vi "VIH Dialog - Search Files in Folder.vi"(8 "error in":errorcluster, 9 "File Paths":path[](array[path]), 10 "Tree Item Tags":string[](array[string]), 11 "Project Tree":T1) -> (0 "error out":errorcluster, 1 "File Paths out":path[](array[path]), 2 "Tree Item Tags out":string[](array[string]), 3 "dup Project Tree":T1)   [LabVIEW 2014]
doc: "::: VI Helpeks :::\nCopyright (c) 2000-2026 Konstantin Shifershteyn. All rights reserved."
uses:
  VIH Project Tree Typedef - Tree Refnum.ctl
panel:
  # "VI Helpeks\nCopyright (c) 2012-2026 Konstantin Shifershteyn"
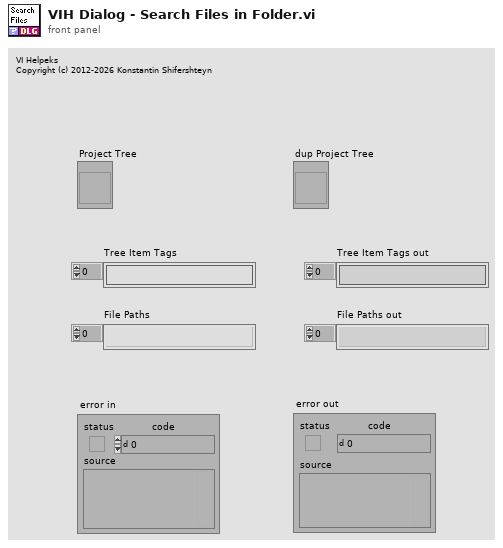
[diagram p1: front panel]
types:
  T1 = typedef "VIH Project Tree Typedef - Tree Refnum.ctl" = refnum<vi>
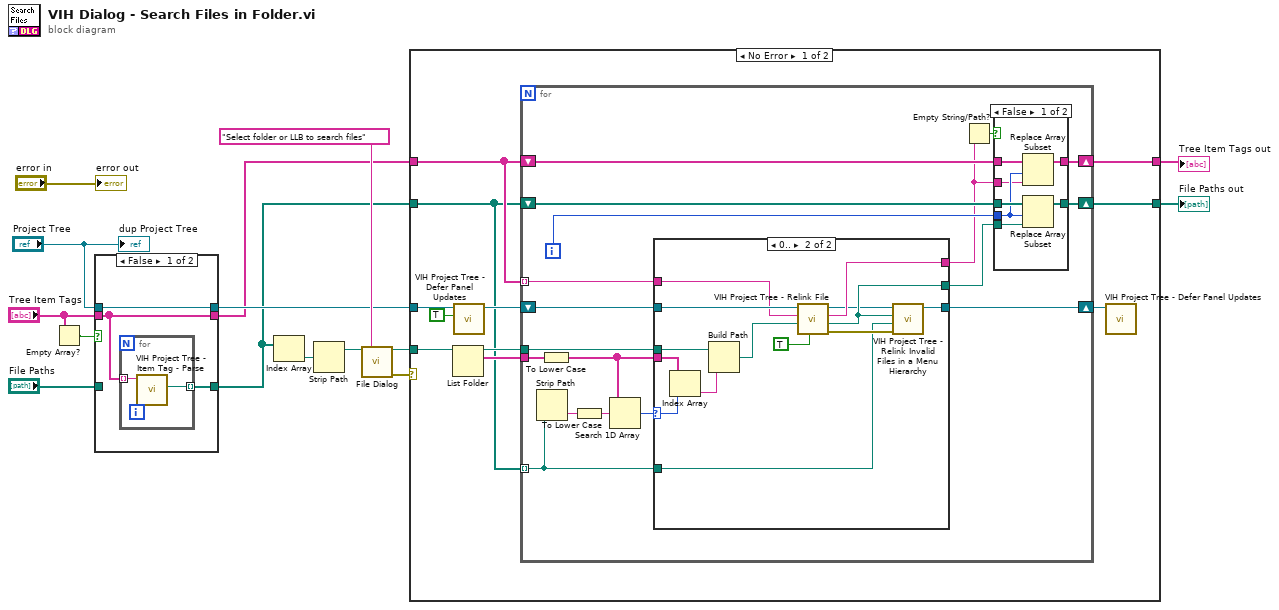
[diagram p0: block diagram]
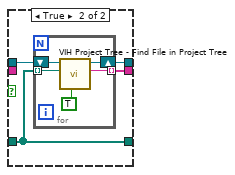
[diagram p2: hidden frame]
diagram:
  n1 = Empty Array?(array="Tree Item Tags") -> (empty?=w10:bool)
  n2 = case shown="False" w10 {
    tunnel: [w18 w24] -> w4
    tunnel: "Tree Item Tags" -> [w18 _]
    tunnel: [w17 w23] -> w3
    tunnel: "File Paths" -> [_ w23]
    tunnel: "Project Tree" -> [w16 w22]
    tunnel: [w16 w21] -> w6
    frame False {
      n3 = for {
        tunnel: w18 -> [w20] mode=indexing
        tunnel: [w19] -> w17 mode=indexing
        n4 = call "VIH Project Tree - Item Tag - Parse.vi"("Tree Item Tag"=w20) -> ("Item File Path"=w19:path)  [unwired: 8 in, 2 out]
      }
    }
    frame True {
      n5 = for {
        tunnel: [w28] -> w24 mode=indexing
        tunnel: w23 -> [w27] mode=indexing
        shift-right: [w25] -> w21
        shift-left: w22 -> [w26]
        n6 = call "VIH Project Tree - Find File in Project Tree.vi"("Ena <Invalid> (F)"=TRUE, "File Path"=w27, "Project Tree"=w26) -> ("Tree Item Tag (Static)"=w28:string, "dup Project Tree"=w25:T1)  [unwired: 5 in, 2 out]
      }
    }
  }
  n7 = Index Array(array=w3) -> (element=w5:path)  [unwired: 1 in]
  n8 = Strip Path(path=w5) -> (stripped path=w14:path)  [unwired: 1 out]
  n9 = call "File Dialog"("start path"=w14, "prompt"="Select folder or LLB to search files") -> ("selected path"=w13:path, "error out"=w12:errorcluster)  [unwired: 10 in, 2 out]
  n10 = case shown="No Error" w12 {
    tunnel: w6 -> [w40 _]
    tunnel: w13 -> [w36 _]
    tunnel: w4 -> [w33 _]
    tunnel: w3 -> [w32 _]
    tunnel: [w31 _] -> w2
    tunnel: [w30 _] -> w1
    frame No Error {
      n11 = List Folder(path=w36) -> (path out=w34:path, filenames=w35:string[])  [unwired: 3 in, 2 out]
      n12 = call "VIH Project Tree - Defer Panel Updates.vi"("Defer Panel Updates (F)"=TRUE, "Project Tree"=w40) -> ("dup Project Tree"=w39:T1)  [unwired: 7 in, 2 out]
      n13 = for {
        tunnel: w32 -> [w56] mode=indexing
        shift-right: [w57] -> w38
        shift-left: w39 -> [w58]
        tunnel: w35 -> [w54]
        tunnel: w33 -> [w52] mode=indexing
        tunnel: w34 -> [w50]
        shift-right: [w46] -> w31
        shift-left: w33 -> [w48]
        shift-right: [w45] -> w30
        shift-left: w32 -> [w47]
        i -> [w44]
        n14 = Strip Path(path=w56) -> (name=w55:string)  [unwired: 1 out]
        n15 = To Lower Case(string=w54) -> (all lower case string=w49:string[])
        n16 = To Lower Case(string=w55) -> (all lower case string=w53:string)
        n17 = Search 1D Array(1D array=w49, element=w53) -> (index of element=w51:i32)  [unwired: 1 in]
        n18 = case shown="0.." w51 {
          selector: w51 -> [_ w71]
          tunnel: [_ w82] -> w43
          tunnel: [_ w81] -> w42
          tunnel: w58 -> [w68 w77]
          tunnel: [w68 w76] -> w57
          tunnel: w56 -> [_ w75]
          tunnel: w52 -> [_ w74]
          tunnel: w50 -> [_ w73]
          tunnel: w49 -> [_ w72]
          frame ..-1 {
          }
          frame 0.. {
            n19 = Index Array(array=w72, index=w71) -> (element=w70:string)
            n20 = Build Path(base path=w73, name or relative path=w70) -> (appended path=w69:path)
            n21 = call "VIH Project Tree - Relink File.vi"("Ena Dialog Message (T)"=TRUE, "New File Path"=w69, "Tree Item Tag"=w74, "Project Tree"=w77) -> ("error out"=w78:errorcluster, "New File Path out"=w81:path, "New Tree Item Tag"=w82:string, "dup Project Tree"=w80:T1)  [unwired: 4 in]
            n22 = call "VIH Project Tree - Relink Invalid Files in a Menu Hierarchy.vi"("error in"=w78, "old Item Path"=w75, "new Item Path"=w81, "Project Tree"=w80) -> ("dup Project Tree"=w76:T1)  [unwired: 6 in, 1 out]
          }
        }
        n23 = Empty String/Path?(string/path=w43) -> (empty?=w41:bool)
        n24 = case shown="False" w41 {
          tunnel: w48 -> [w65 w67]
          tunnel: w47 -> [w64 w66]
          tunnel: [w63 w67] -> w46
          tunnel: [w62 w66] -> w45
          tunnel: w44 -> [w61 _]
          tunnel: w43 -> [w60 _]
          tunnel: w42 -> [w59 _]
          frame False {
            n25 = Replace Array Subset(array=w65, new element=w60, index=w61) -> (w63:string[])
            n26 = Replace Array Subset(array=w64, new element=w59, index=w61) -> (w62:path[])
          }
          frame True {
          }
        }
      }
      n27 = call "VIH Project Tree - Defer Panel Updates.vi"("Project Tree"=w38) -> ()  [unwired: 8 in, 3 out]
    }
    frame Error {
    }
  }
  "Tree Item Tags out" <- w2
  "File Paths out" <- w1
  "dup Project Tree" <- "Project Tree"
  "error out" <- "error in"
